vi "Tool Object.vi"(8 "error in (no error)":errorcluster, 11 "Tool Path in":refnum<class "Tool Path.lvclass">) -> (0 "error out":errorcluster, 3 "Tool Path out":refnum<class "Tool Path.lvclass">)   [LabVIEW 2019, in "Tool Path.lvclass"]
uses:
  Tool Path.lvclass
  Settings/ObjectSettings/ObjectSettings.lvclass
  Parse/PathCommands/Point.ctl
  Parse/PathCommands/PathCommands.lvclass
  Tool Object/Tool Object.lvclass
  Parse/ParsePaths/Path.lvclass
  Settings/Path Settings/Path Settings.lvclass
  C:/Users/Albro/Documents/GitHub/AFM-Lithography/lvsrc/Classes/Tool/Tool Object/Tool Object.lvclass
  C:/Users/Albro/Documents/GitHub/AFM-Lithography/lvsrc/Classes/Settings/ObjectSettings/ObjectSettings.lvclass
panel:
  out "All":u32
  out "Make CMD Abs":u32
  out "Get Needed":u32
  out "Apply Trans":u32
  out "Get Path Points":u32
  out "Apply Settings":u32
  out "Path Deviation":u32
  out "Remove Duplicates":u32
  out "Generating Path Points":u32
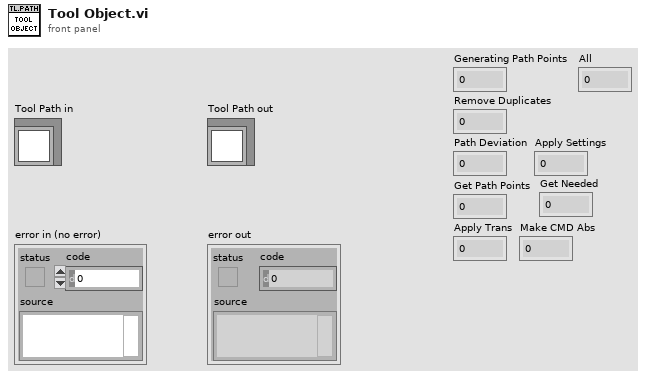
[diagram p1: front panel]
types:
  T1 = typedef "PathCommands.lvclass/Point.ctl" = cluster{"X":dbl, "Y":dbl}
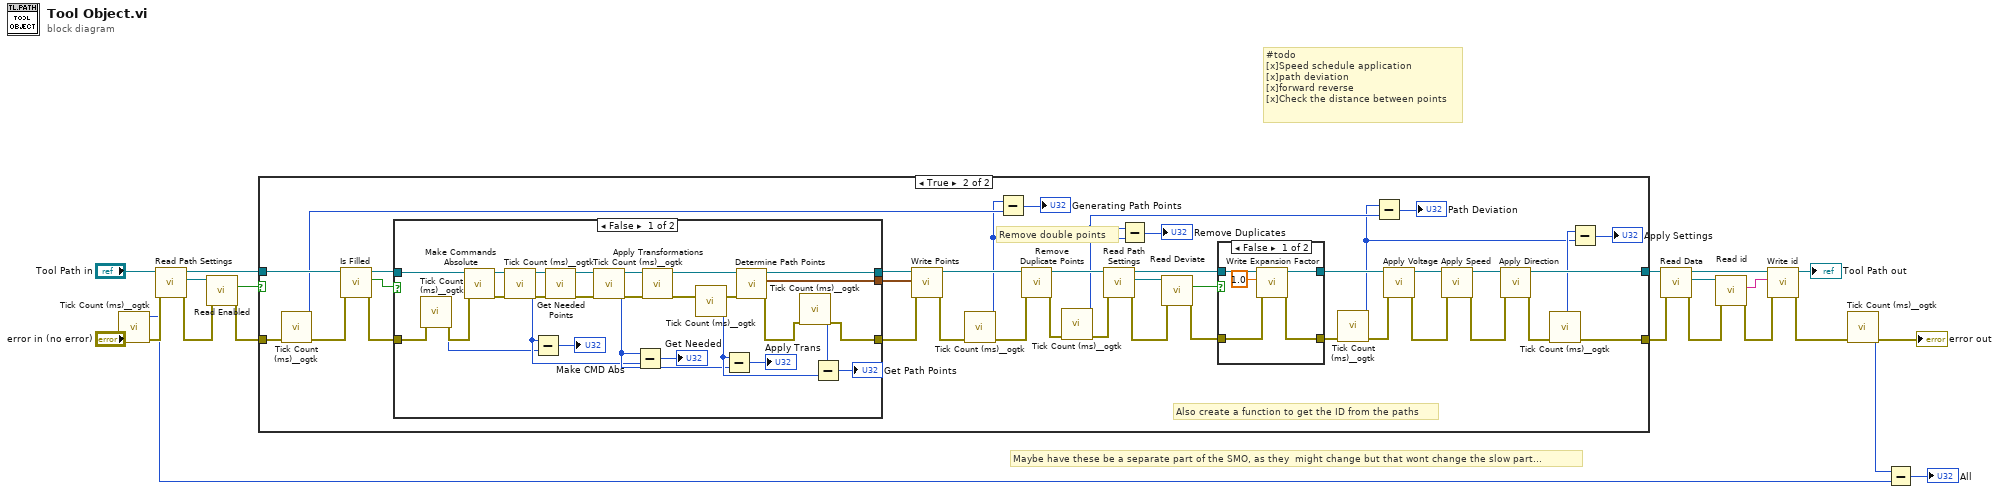
[diagram p0: block diagram]
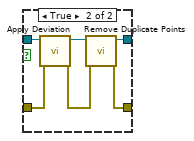
[diagram p3: hidden frame]
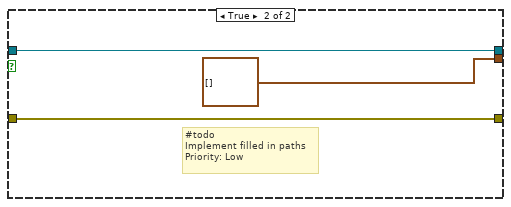
[diagram p4: hidden frame]
diagram:
  # "Maybe have these be a separate part of the SMO, as they  might change but that wont change the slow part..."
  # "#todo\n[x]Speed schedule application\n[x]path deviation\n[x]forward reverse\n[x]Check the distance between points"
  n1 = call <userlib>:"Tick Count (ms)__ogtk.vi"("error in (no error)"="error in (no error)") -> ("error out"=w5:errorcluster, "millisecond timer value"=w2:u32)  [unwired: 9 in]
  n2 = call-dynamic "Read Path Settings.vi"("error in (no error)"=w5, "Tool Path in"="Tool Path in") -> ("error out"=w16:errorcluster, "Path Settings.lvclass"=w20:refnum<class "Path Settings.lvclass">, "Tool Path out"=w19:refnum<class "Tool Path.lvclass">)  [unwired: 7 in]
  n3 = call "Read Enabled.vi"("error in (no error)"=w16, "ObjectSettings in"=w20) -> ("error out"=w15:errorcluster, "Enabled"=w18:bool)  [unwired: 7 in, 1 out]
  n4 = case shown="True" w18 {
    tunnel: w19 -> [w23 w61]
    tunnel: [w23 w41] -> w9
    tunnel: w15 -> [w22 w34]
    tunnel: [w22 w36] -> w7
    frame False {
    }
    frame True {
      # "Also create a function to get the ID from the paths"
      # "Remove double points"
      n5 = call <userlib>:"Tick Count (ms)__ogtk.vi"("error in (no error)"=w34) -> ("error out"=w35:errorcluster, "millisecond timer value"=w33:u32)  [unwired: 9 in]
      n6 = call "Is Filled.vi"("error in (no error)"=w35, "Tool Path in"=w61) -> ("error out"=w59:errorcluster, "Filled?"=w60:bool, "Tool Path out"=w62:refnum<class "Tool Path.lvclass">)  [unwired: 7 in]
      n7 = case shown="False" w60 {
        tunnel: w62 -> [w95 w101]
        tunnel: [w98 w101] -> w58
        tunnel: w59 -> [w89 w100]
        tunnel: [w83 w100] -> w57
        tunnel: [w97 T1[] [] ("Points")] -> w24
        frame False {
          n8 = call <userlib>:"Tick Count (ms)__ogtk.vi"("error in (no error)"=w89) -> ("error out"=w90:errorcluster, "millisecond timer value"=w75:u32)  [unwired: 9 in]
          n9 = call "Make Commands Absolute.vi"("error in (no error)"=w90, "Tool Path in"=w95) -> ("error out"=w93:errorcluster, "Tool Path out"=w94:refnum<class "Tool Path.lvclass">)  [unwired: 8 in]
          n10 = call <userlib>:"Tick Count (ms)__ogtk.vi"("error in (no error)"=w93) -> ("error out"=w88:errorcluster, "millisecond timer value"=w76:u32)  [unwired: 9 in]
          n11 = Subtract(x=w76, y=w75) -> (x-y=→"Make CMD Abs":u32)
          n12 = call-dynamic "Get Needed Points.vi"("error in (no error)"=w88, "Tool Path in"=w94) -> ("error out"=w92:errorcluster, "Tool Path out"=w91:refnum<class "Tool Path.lvclass">)  [unwired: 8 in]
          n13 = call <userlib>:"Tick Count (ms)__ogtk.vi"("error in (no error)"=w92) -> ("error out"=w87:errorcluster, "millisecond timer value"=w78:u32)  [unwired: 9 in]
          n14 = Subtract(x=w78, y=w76) -> (x-y=→"Get Needed":u32)
          n15 = call-dynamic "Apply Transformations.vi"("error in (no error)"=w87, "Tool Path in"=w91) -> ("error out"=w86:errorcluster, "Tool Path out"=w96:refnum<class "Tool Path.lvclass">)  [unwired: 8 in]
          n16 = call <userlib>:"Tick Count (ms)__ogtk.vi"("error in (no error)"=w86) -> ("error out"=w85:errorcluster, "millisecond timer value"=w80:u32)  [unwired: 9 in]
          n17 = Subtract(x=w80, y=w78) -> (x-y=→"Apply Trans":u32)
          n18 = call-dynamic "Determine Path Points.vi"("error in (no error)"=w85, "Tool Path in"=w96) -> ("error out"=w84:errorcluster, "Points"=w97:T1[], "Tool Path out"=w98:refnum<class "Tool Path.lvclass">)  [unwired: 7 in]
          n19 = call <userlib>:"Tick Count (ms)__ogtk.vi"("error in (no error)"=w84) -> ("error out"=w83:errorcluster, "millisecond timer value"=w82:u32)  [unwired: 9 in]
          n20 = Subtract(x=w82, y=w80) -> (x-y=→"Get Path Points":u32)
        }
        frame True {
          # "#todo\nImplement filled in paths\nPriority: Low"
        }
      }
      n21 = call-dynamic "Write Points.vi"("error in (no error)"=w57, "Points"=w24, "Tool Object in"=w58) -> ("error out"=w51:errorcluster, "Tool Object out"=w56:refnum<class "Tool Path.lvclass">)  [unwired: 7 in]
      n22 = call <userlib>:"Tick Count (ms)__ogtk.vi"("error in (no error)"=w51) -> ("error out"=w39:errorcluster, "millisecond timer value"=w31:u32)  [unwired: 9 in]
      n23 = Subtract(x=w31, y=w33) -> (x-y=→"Generating Path Points":u32)
      n24 = call "Remove Duplicate Points.vi"("error in (no error)"=w39, "Tool Object in"=w56) -> ("error out"=w49:errorcluster, "Tool Object out"=w44:refnum<class "Tool Path.lvclass">)  [unwired: 8 in]
      n25 = call <userlib>:"Tick Count (ms)__ogtk.vi"("error in (no error)"=w49) -> ("error out"=w38:errorcluster, "millisecond timer value"=w29:u32)  [unwired: 9 in]
      n26 = call-dynamic "Read Path Settings.vi"("error in (no error)"=w38, "Tool Path in"=w44) -> ("error out"=w53:errorcluster, "Path Settings.lvclass"=w54:refnum<class "Path Settings.lvclass">, "Tool Path out"=w55:refnum<class "Tool Path.lvclass">)  [unwired: 7 in]
      n27 = Subtract(x=w29, y=w31) -> (x-y=→"Remove Duplicates":u32)
      n28 = call-dynamic "Read Deviate.vi"("error in (no error)"=w53, "Path Settings in"=w54) -> ("error out"=w50:errorcluster, "Deviate"=w52:bool)  [unwired: 7 in, 1 out]
      n29 = case shown="False" w52 {
        tunnel: [w67 w71] -> w43
        tunnel: [w64 w68] -> w42
        tunnel: w55 -> [w66 w72]
        tunnel: w50 -> [w63 w73]
        frame False {
          n30 = call-dynamic "Write Expansion Factor.vi"("error in (no error)"=w63, "Expansion Factor"=1.0, "Tool Path in"=w66) -> ("error out"=w64:errorcluster, "Tool Path out"=w67:refnum<class "Tool Path.lvclass">)  [unwired: 7 in]
        }
        frame True {
          n31 = call-dynamic "Apply Deviation.vi"("error in (no error)"=w73, "Tool Path in"=w72) -> ("error out"=w69:errorcluster, "Tool Path out"=w70:refnum<class "Tool Path.lvclass">)  [unwired: 8 in]
          n32 = call "Remove Duplicate Points.vi"("error in (no error)"=w69, "Tool Object in"=w70) -> ("error out"=w68:errorcluster, "Tool Object out"=w71:refnum<class "Tool Path.lvclass">)  [unwired: 8 in]
        }
      }
      n33 = call <userlib>:"Tick Count (ms)__ogtk.vi"("error in (no error)"=w42) -> ("error out"=w37:errorcluster, "millisecond timer value"=w26:u32)  [unwired: 9 in]
      n34 = Subtract(x=w26, y=w29) -> (x-y=→"Path Deviation":u32)
      n35 = call-dynamic "Apply Voltage.vi"("error in (no error)"=w37, "Tool Path in"=w43) -> ("error out"=w47:errorcluster, "Tool Path out"=w48:refnum<class "Tool Path.lvclass">)  [unwired: 8 in]
      n36 = call-dynamic "Apply Speed.vi"("error in (no error)"=w47, "Tool Path in"=w48) -> ("error out"=w46:errorcluster, "Tool Path out"=w45:refnum<class "Tool Path.lvclass">)  [unwired: 8 in]
      n37 = call-dynamic "Apply Direction.vi"("error in (no error)"=w46, "Tool Path in"=w45) -> ("error out"=w40:errorcluster, "Tool Path out"=w41:refnum<class "Tool Path.lvclass">)  [unwired: 8 in]
      n38 = call <userlib>:"Tick Count (ms)__ogtk.vi"("error in (no error)"=w40) -> ("error out"=w36:errorcluster, "millisecond timer value"=w27:u32)  [unwired: 9 in]
      n39 = Subtract(x=w27, y=w26) -> (x-y=→"Apply Settings":u32)
    }
  }
  n40 = call-dynamic "Read Data.vi"("error in (no error)"=w7, "Tool Path in"=w9) -> ("error out"=w11:errorcluster, "Path.lvclass"=w14:refnum<class "Path.lvclass">, "Tool Path out"=w13:refnum<class "Tool Path.lvclass">)  [unwired: 7 in]
  n41 = call-dynamic "Read id.vi"("error in (no error)"=w11, "SVG Object in"=w14) -> ("error out"=w10:errorcluster, "id"=w12:string)  [unwired: 7 in, 1 out]
  n42 = call-dynamic "Write id.vi"("error in (no error)"=w10, "id"=w12, "Tool Path in"=w13) -> ("error out"=w6:errorcluster, "Tool Path out"=→"Tool Path out":refnum<class "Tool Path.lvclass">)  [unwired: 7 in]
  n43 = call <userlib>:"Tick Count (ms)__ogtk.vi"("error in (no error)"=w6) -> ("error out"=→"error out":errorcluster, "millisecond timer value"=w3:u32)  [unwired: 9 in]
  n44 = Subtract(x=w3, y=w2) -> (x-y=→"All":u32)
